vi "GET-Version.vi"(8 "error in (no error)":errorcluster, 10 "ApiKey":string, 11 "BaseUrl":string) -> (0 "error out":errorcluster, 3 "Version":cluster{"version":string})   [LabVIEW 2017]
uses:
  <vilib>/httpClient/LabVIEWHTTPClient.lvlib
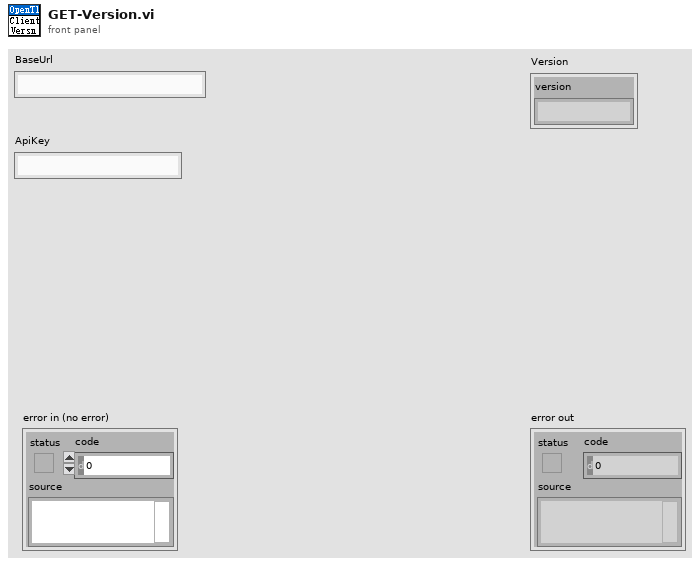
[diagram p1: front panel]
types:
  T1 = typedef "LabVIEWHTTPClient.lvlib/ClientHandle.ctl" = refnum<k1>
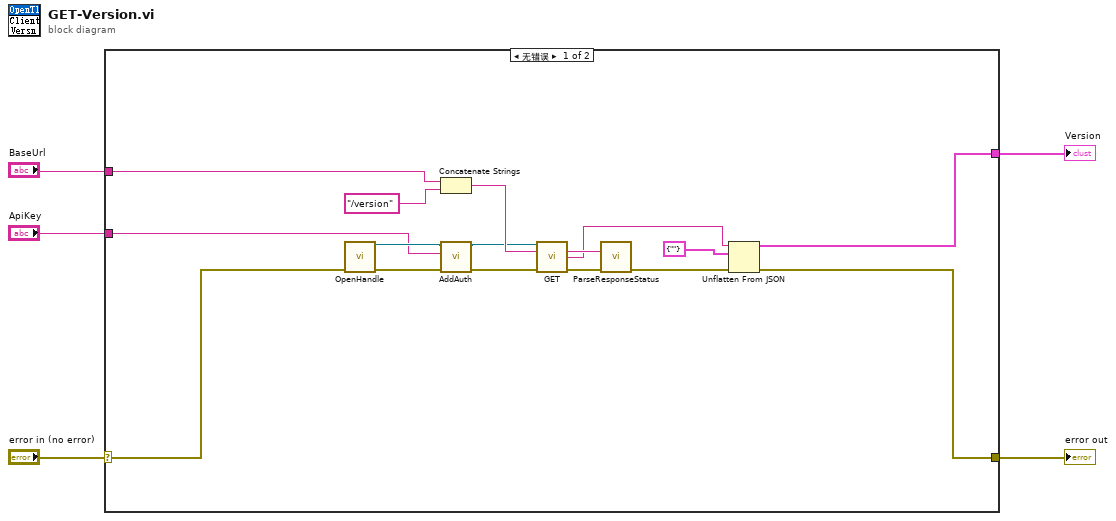
[diagram p0: block diagram]
diagram:
  n1 = case shown="无错误" "error in (no error)" {
    selector: "error in (no error)" -> [w16 w22]
    tunnel: [w18 w22] -> w4
    tunnel: [w19 _] -> w3
    tunnel: "BaseUrl" -> [w17 _]
    tunnel: "ApiKey" -> [w11 _]
    frame No Error {
      n2 = call <vilib>:"OpenHandle.vi"("error in (no error)"=w16) -> ("client handle out"=w15:T1, "error out"=w14:errorcluster)  [unwired: 13 in]
      n3 = Concatenate Strings(w17, "/version" ("url")) -> (w20:string)
      n4 = call "AddAuth.vi"("error in (no error)"=w14, "ApiKey"=w11, "client handle in"=w15) -> ("error out"=w13:errorcluster, "client handle out"=w12:T1)  [unwired: 7 in]
      n5 = call <vilib>:"GET.vi"("client handle"=w12, "url"=w20, "error in (no error)"=w13) -> ("headers"=w10:string, "body"=w6:string, "error out"=w9:errorcluster)  [unwired: 9 in, 1 out]
      n6 = call "ParseResponseStatus.vi"("error in (no error)"=w9, "Headers"=w10) -> ("error out"=w8:errorcluster)  [unwired: 7 in, 2 out]
      n7 = Unflatten From JSON(JSON string=w6, type and defaults=cluster{"version":string} {"version"=""} ("Version"), error in (no error)=w8) -> (value=w19:cluster{"version":string}, error out=w18:errorcluster)  [unwired: 4 in]
    }
    frame Error {
    }
  }
  "error out" <- w4
  "Version" <- w3
